vi "AMR_Status.vi"(8 "error in (no error)":errorcluster caption="에러 입력(에러 없음)", 11 "Robot-AMR 2":T1) -> (0 "error out":errorcluster caption="에러 출력", 2 "Level":dbl, 3 "Vx":dbl)   [LabVIEW 2019]
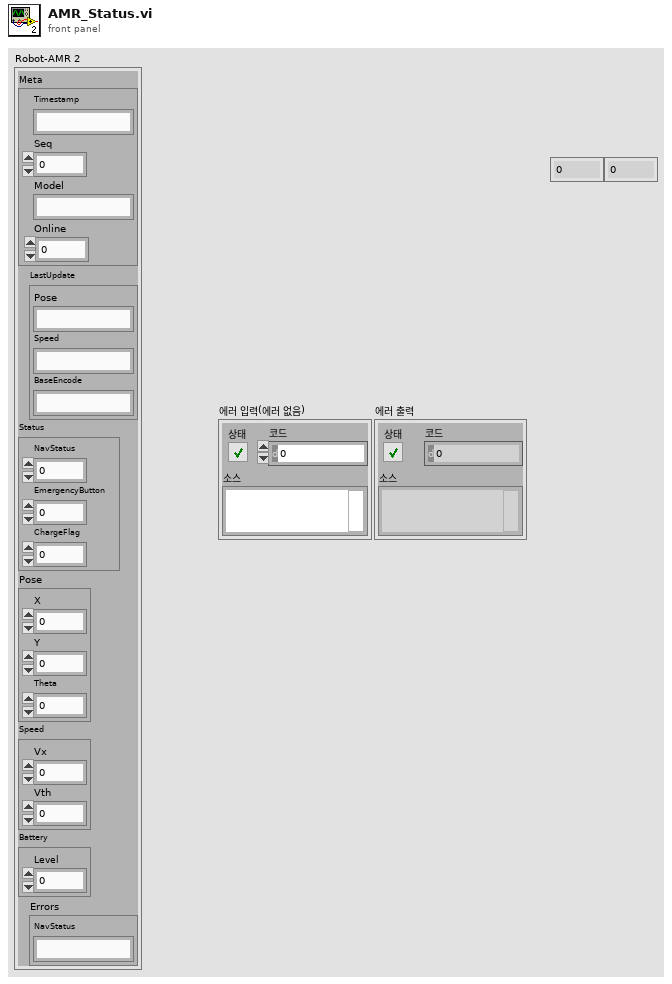
[diagram p1: front panel]
types:
  T1 = cluster{"Meta":cluster{"Timestamp":string, "Seq":dbl, "Model":string, "Online":dbl}, "LastUpdate":cluster{"Pose":string, "Speed":string, "BaseEncode":string}, "Status":cluster{"NavStatus":dbl, "EmergencyButton":dbl, "ChargeFlag":dbl}, "Pose":cluster{"X":dbl, "Y":dbl, "Theta":dbl}, "Speed":cluster{"Vx":dbl, "Vth":dbl}, "Battery":cluster{"Level":dbl}, "Errors":cluster{"NavStatus":string}}
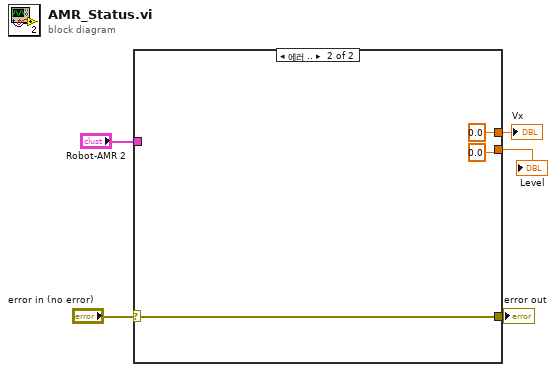
[diagram p0: block diagram]
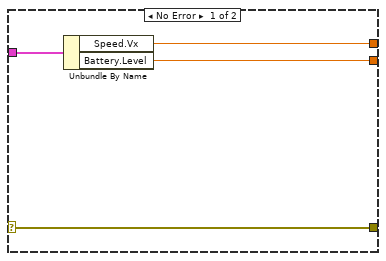
[diagram p2: hidden frame]
diagram:
  n1 = case shown="에러 .." "error in (no error)" {
    selector: "error in (no error)" -> [w9 w12]
    tunnel: [w9 w12] -> w4
    tunnel: "Robot-AMR 2" -> [w8 _]
    tunnel: [w7 0.0 ("Vx")] -> w2
    tunnel: [w6 0.0 ("Level")] -> w1
    frame No Error {
      n2 = Unbundle By Name(w8) -> ("Speed.Vx"=w7:dbl, "Battery.Level"=w6:dbl)
    }
    frame Error {
    }
  }
  "error out" <- w4
  "Vx" <- w2
  "Level" <- w1
